vi "OwnLibrary20261013_Create.vi"() -> ()   [LabVIEW 2024]
panel:
  out "error out":errorcluster caption="错误输出"
  in  "Save Library Path":path
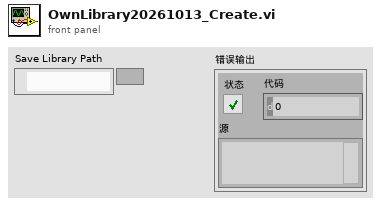
[diagram p1: front panel]
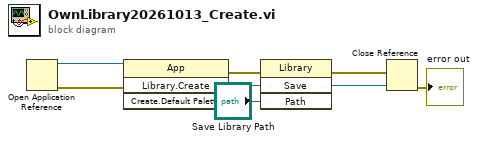
[diagram p0: block diagram]
diagram:
  n1 = Open Application Reference() -> (0:w6:errorcluster, 3:w7:refnum<vi>)  [unwired: 4 in]
  n2 = invoke class="App" method="Library.Create"(reference=w7, error in=w6) -> (error out=w3:errorcluster, "Create Library"=w5:refnum<vi>)  [unwired: 2 in, 2 out]
  n3 = invoke class="Library" method="Save"(reference=w5, error in=w3, "Path"="Save Library Path") -> (error out=w2:errorcluster)  [unwired: 1 in, 3 out]
  n4 = Close Reference(reference=w5, error in (no error)=w2) -> (error out=→"error out":errorcluster)
